vi "Actor Core.vi"(8 "error in (no error)":errorcluster, 11 "Operator UI.lvclass":refnum<class "Measurement UI.lvclass">) -> (0 "error out":errorcluster, 3 "Actor Framework.lvlib:Actor":refnum<class "Actor.lvclass">)   [LabVIEW 2017, in "Measurement UI.lvlib" / "Measurement UI.lvclass"]
doc: "This is Actor Core.vi, the main message handling loop for Actors. An actor usually just sits in this loop and processes messages as they arrive. Any error returned by the message Do.vi call will stop the loop, with error code 43 as the cannonical signal to stop with no error sent to caller. Descendants may override that in Handle Error.vi."
uses:
  Measurement UI.lvclass
  <vilib>/ActorFramework/Actor/Actor.lvclass
  \\Mac\Home/Documents/MAL-Framework/user.lib/Common Components/User Interface/UI.lvclass
  C:/Program Files (x86)/National Instruments/LabVIEW 2017/vi.lib/ActorFramework/Actor/Actor.lvclass
  <vilib>/ActorFramework/Actor/Actor.lvclass/Actor.ctl
  <vilib>/ActorFramework/Message Enqueuer/Message Enqueuer.lvclass/Message Enqueuer.ctl
  <vilib>/ActorFramework/Message Enqueuer/Init from Existing Queue.vi
  <vilib>/ActorFramework/Message Enqueuer/Enqueue.vi
  <vilib>/ActorFramework/Stop Msg/Stop Msg.lvclass
  C:/Program Files (x86)/National Instruments/LabVIEW 2017/vi.lib/ActorFramework/Message/Message.lvclass
  Messages/Ask Controller to Launch Results UI Msg/Ask Controller to Launch Results UI Msg.lvclass
  Measurement UI Messages/Launch Step Configuration Msg/Launch Step Configuration Msg.lvclass
  Accessors/Write Digitizer.vi
  Accessors/Write Function Generator.vi
  Accessors/Write Load New Measurement.vi
  Accessors/Write Measurement.vi
  Accessors/Write Multimeter.vi
  Accessors/Write Power Supply.vi
  Accessors/Write Results Listbox.vi
  Accessors/Write Run.vi
  Accessors/Write Show FP_.vi
  Accessors/Write Status Display.vi
  Accessors/Write Stop Button.vi
  Accessors/Write Tab Control.vi
  Accessors/Write View Results.vi
  Write Step Iterations.vi
  Write settings button array for hardware.vi
  Accessors/Write Step Config.vi
  <vilib>/ActorFramework/Message Priority Queue/Priority Enqueue.vi
  <vilib>/ActorFramework/Message Enqueuer/Message Enqueuer.lvclass
  User Interface/UI.lvclass
  Messages/Send Run Measurement Message/Send Run Measurement Message.lvclass
  Messages/Send Get Hardware Info Message/Send Get Hardware Info Message.lvclass
  Messages/Check Run Button/Check Validity of Selection.lvclass
  Messages/Prompt User for Path to load/Prompt User for File Path to Load From.lvclass
  Measurement UI Messages/Launch Hardware Settings Msg/Launch Hardware Settings Msg.lvclass
panel:
  in  "Step Config":bool
  in  "3":bool
  in  "2":bool
  in  "1":bool
  in  "0":bool
  in  "Step Iterations":i32
  in  "Indefinite run":bool
  in  "about":bool
  in  "Load New Measurement":bool
  in  "Show FP?":bool
  in  "Stop Button":bool
  in  "Run":bool
  in  "Device 4":u16(ring)
  in  "Device 3":u16(ring)
  in  "Device 2":u16(ring)
  in  "Device 1":u16(ring)
  in  "Tab Control":enum32{"Test Status", "Results"}(tab)
  in  "Status Display":string
  in  "View Results":bool
  in  "Results Listbox":i32(listbox)
  in  "Step":u16(ring)
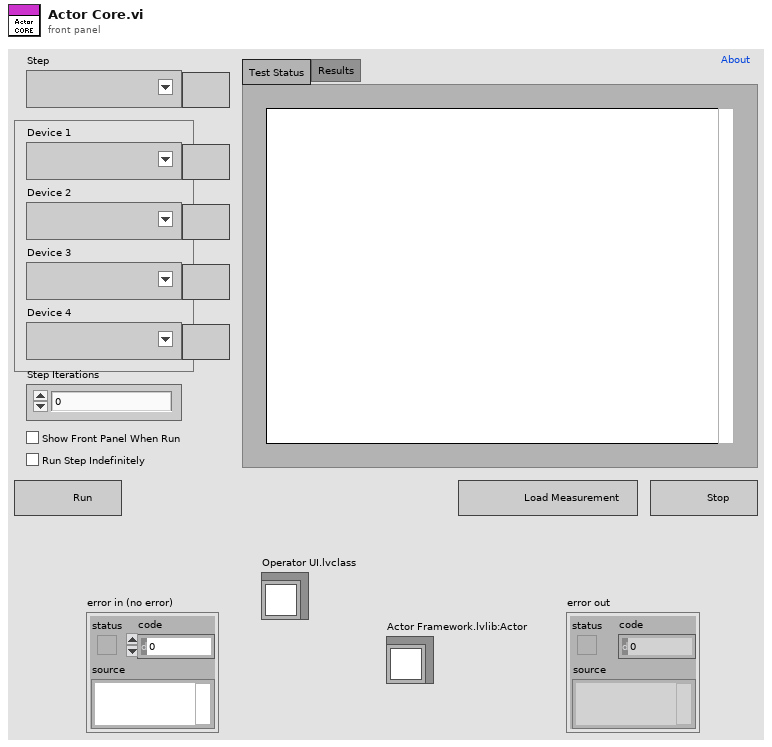
[diagram p1: front panel]
types:
  T1 = enum8{"Enabled", "Disabled", "Disabled and Grayed Out"}
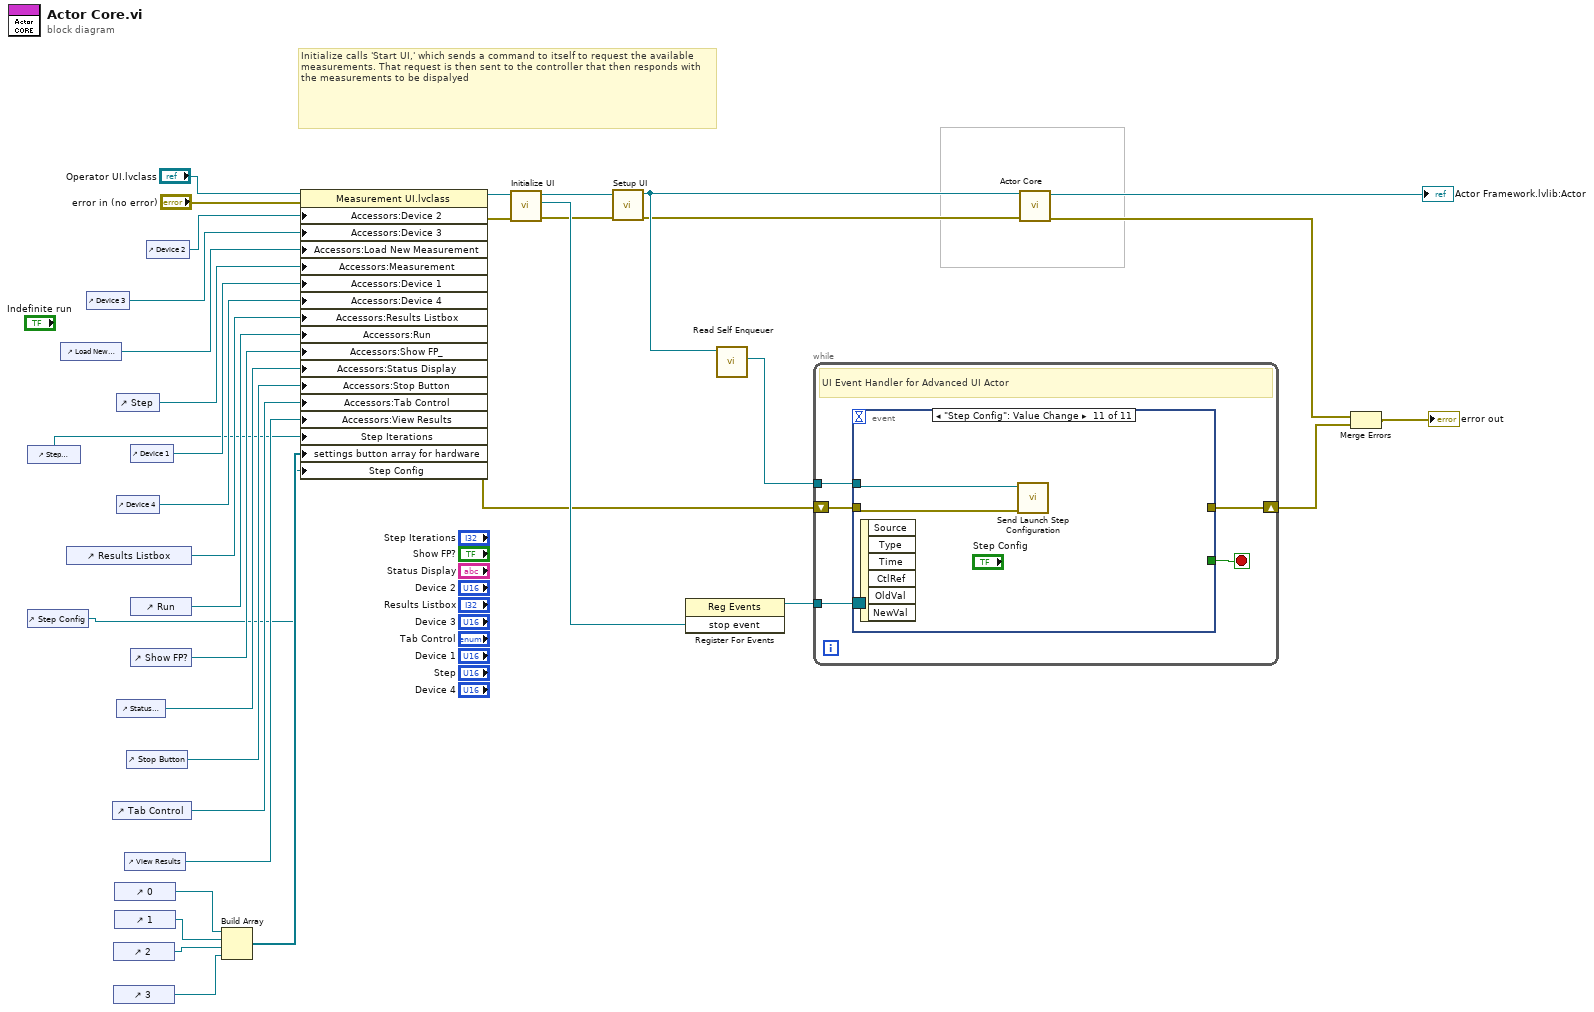
[diagram p0: block diagram]
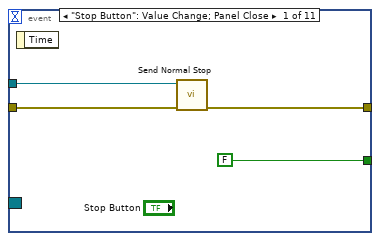
[diagram p2: hidden frame]
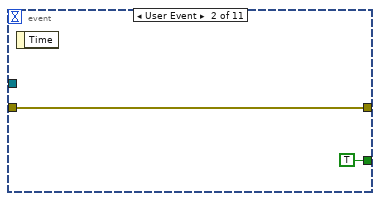
[diagram p3: hidden frame]
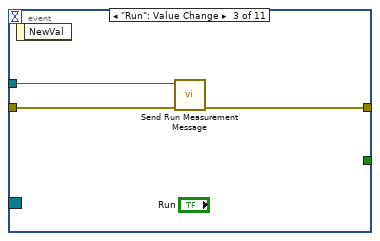
[diagram p4: hidden frame]
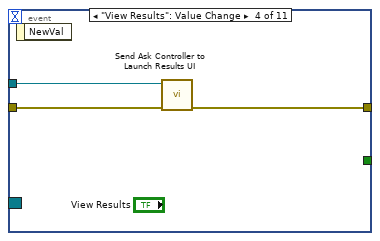
[diagram p5: hidden frame]
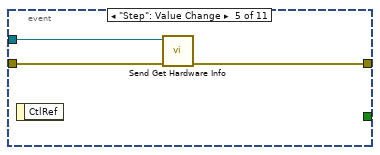
[diagram p6: hidden frame]
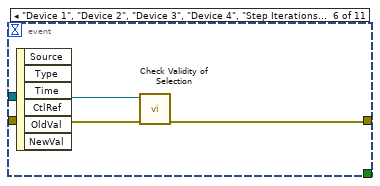
[diagram p7: hidden frame]
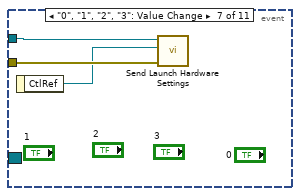
[diagram p8: hidden frame]
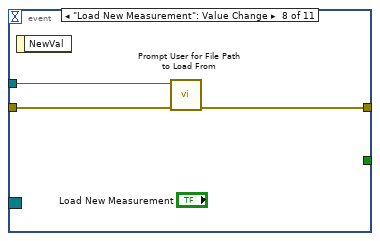
[diagram p9: hidden frame]
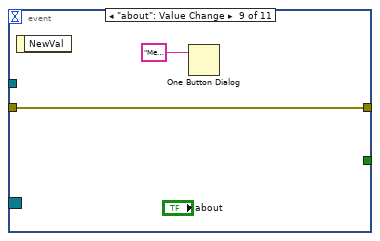
[diagram p10: hidden frame]
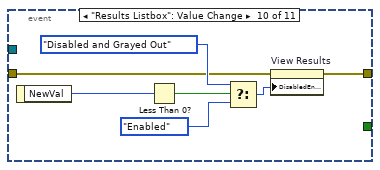
[diagram p11: hidden frame]
diagram:
  # "Initialize calls 'Start UI,' which sends a command to itself to request the available measurements. That request is then sent to the controller that then responds with the measurements to be dispalyed"
  n1 = control-ref of="Step Iterations"() -> (w7:refnum<vi>)
  n2 = control-ref of="Step Config"() -> (w1:refnum<vi>)
  n3 = control-ref of="Load New Measurement"() -> (w18:refnum<vi>)
  n4 = control-ref of="Results Listbox"() -> (w22:refnum<vi>)
  n5 = control-ref of="Device 3"() -> (w19:refnum<vi>)
  n6 = control-ref of="Tab Control"() -> (w24:refnum<vi>)
  n7 = control-ref of="2"() -> (w4:refnum<vi>)
  n8 = control-ref of="3"() -> (w3:refnum<vi>)
  n9 = control-ref of="0"() -> (w6:refnum<vi>)
  n10 = control-ref of="1"() -> (w5:refnum<vi>)
  n11 = control-ref of="Step"() -> (w17:refnum<vi>)
  n12 = control-ref of="Device 4"() -> (w21:refnum<vi>)
  n13 = control-ref of="Status Display"() -> (w26:refnum<vi>)
  n14 = control-ref of="View Results"() -> (w23:refnum<vi>)
  n15 = control-ref of="Stop Button"() -> (w25:refnum<vi>)
  n16 = control-ref of="Device 1"() -> (w16:refnum<vi>)
  n17 = control-ref of="Run"() -> (w15:refnum<vi>)
  n18 = control-ref of="Show FP?"() -> (w27:refnum<vi>)
  n19 = control-ref of="Device 2"() -> (w20:refnum<vi>)
  n20 = Build Array(w6, w5, w4, w3) -> (w2:refnum<vi>[])
  n21 = property class="Measurement UI.lvclass"(reference="Operator UI.lvclass", error in="error in (no error)", "Accessors:Device 2"=w20, "Accessors:Device 3"=w19, "Accessors:Load New Measurement"=w18, "Accessors:Measurement"=w17, "Accessors:Device 1"=w16, "Accessors:Device 4"=w21, "Accessors:Results Listbox"=w22, "Accessors:Run"=w15, "Accessors:Show FP_"=w27, "Accessors:Status Display"=w26, "Accessors:Stop Button"=w25, "Accessors:Tab Control"=w24, "Accessors:View Results"=w23, "Step Iterations"=w7, "settings button array for hardware"=w2, "Step Config"=w1) -> (reference out=w13:refnum<class "Measurement UI.lvclass">, error out=w10:errorcluster)
  n22 = call "Initialize UI.vi"("error in (no error)"=w10, "UI in"=w13) -> ("error out"=w11:errorcluster, "stop event"=w29:refnum<user-event>, "UI out"=w12:refnum<class "Measurement UI.lvclass">)  [unwired: 7 in]
  n23 = call-dynamic "Setup UI.vi"("error in (no error)"=w11, "Operator UI in"=w12) -> ("error out"=w8:errorcluster, "Operator UI out"=w9:refnum<class "Measurement UI.lvclass">)  [unwired: 8 in]
  n24 = register-events(w29) -> (reference out=w30:refnum<event-registration>)  [unwired: 2 in, 1 out]
  n25 = call <vilib>:"Read Self Enqueuer.vi"("Actor"=w9) -> ("Self Enqueuer"=w34:refnum<class "Message Enqueuer.lvclass">)  [unwired: 10 in]
  n26 = while {
    tunnel: w34 -> [w39]
    tunnel: w30 -> [w38]
    shift-right: [w36] -> w33
    shift-left: w10 -> [w37]
    stop <- w40 stop-if-true
    # "UI Event Handler for Advanced UI Actor"
    n27 = event shown="[10] \"Step Config\": Value Change" {
      selector: w38 -> [_ _ _ _ _ _ _ _ _ _ _]
      dyn-events: _ -> [_ _ _ _ _ _ _ _ _ _ _]
      timeout: _ -> [_ _ _ _ _ _ _ _ _ _ _]
      tunnel: [FALSE TRUE _ _ _ _ _ _ _ _ _] -> w40
      tunnel: w39 -> [w43 _ w49 w52 w55 w58 w61 w64 _ _ w75]
      tunnel: w37 -> [w42 w45 w48 w51 w54 w57 w60 w63 w65 w68 w74]
      tunnel: [w41 w45 w47 w50 w53 w56 _ w62 w65 w67 _] -> w36
      event "Stop Button": Value Change; Panel Close {
        n28 = event-data() -> ()  [unwired: 1 in, 1 out]
        n29 = call <vilib>:"Send Normal Stop.vi"("error in (no error)"=w42, "Message Enqueuer"=w43) -> ("error out"=w41:errorcluster)  [unwired: 9 in]
      }
      event User Event {
        n30 = event-data() -> ()  [unwired: 1 in, 1 out]
      }
      event "Run": Value Change {
        n31 = event-data() -> ()  [unwired: 1 in, 1 out]
        n32 = call "Send Run Measurement Message.vi"("error in (no error)"=w48, "Message Enqueuer in"=w49) -> ("error out"=w47:errorcluster)  [unwired: 8 in, 1 out]
      }
      event "View Results": Value Change {
        n33 = event-data() -> ()  [unwired: 1 in, 1 out]
        n34 = call "Send Ask Controller to Launch Results UI.vi"("error in (no error)"=w51, "Message Enqueuer in"=w52) -> ("error out"=w50:errorcluster)  [unwired: 8 in, 1 out]
      }
      event "Step": Value Change {
        n35 = event-data() -> ()  [unwired: 1 in, 1 out]
        n36 = call "Send Get Hardware Info.vi"("error in (no error)"=w54, "Message Enqueuer in"=w55) -> ("error out"=w53:errorcluster)  [unwired: 8 in, 1 out]
      }
      event "Device 1", "Device 2", "Device 3", "Device 4", "Step Iterations", "Indefinite run": Value Change {
        n37 = event-data() -> ()  [unwired: 1 in, 6 out]
        n38 = call "Check Validity of Selection.vi"("error in (no error)"=w57, "Message Enqueuer in"=w58) -> ("error out"=w56:errorcluster)  [unwired: 8 in, 1 out]
      }
      event "0", "1", "2", "3": Value Change {
        n39 = event-data() -> ("CtlRef"=w59:refnum<vi>)  [unwired: 1 in]
        n40 = call "Send Launch Hardware Settings.vi"("error in (no error)"=w60, "button ref"=w59, "Message Enqueuer"=w61) -> ()  [unwired: 7 in, 2 out]
      }
      event "Load New Measurement": Value Change {
        n41 = event-data() -> ()  [unwired: 1 in, 1 out]
        n42 = call "Prompt User for File Path to Load From.vi"("error in (no error)"=w63, "Message Enqueuer in"=w64) -> ("error out"=w62:errorcluster)  [unwired: 8 in, 1 out]
      }
      event "about": Value Change {
        n43 = event-data() -> ()  [unwired: 1 in, 1 out]
        n44 = One Button Dialog(message="Measurement Manager v2.0\n\nNational Instruments (C) 2013\nWritten in NI LabVIEW 2012 by Elijah Kerry \nElijah.Kerry@ni.com\n\nni.com/largeapps\nekerry.wordpress.com") -> ()  [unwired: 1 in, 1 out]
      }
      event "Results Listbox": Value Change {
        n45 = event-data() -> ("NewVal"=w69:i32)  [unwired: 1 in]
        n46 = Less Than 0?(x=w69) -> (x < 0?=w70:bool)
        n47 = Select(t=T1."Disabled and Grayed Out" ("Disabled"), s=w70, f=T1."Enabled" ("Disabled")) -> (s? t:f=w73:T1)
        n48 = property on="View Results" class="Bool"(error in=w68, "DisabledEnum"=w73) -> (error out=w67:errorcluster)  [unwired: 1 in, 1 out]
      }
      event "Step Config": Value Change {
        n49 = event-data() -> ()  [unwired: 1 in, 6 out]
        n50 = call "Send Launch Step Configuration.vi"("error in (no error)"=w74, "Message Enqueuer"=w75) -> ()  [unwired: 8 in, 2 out]
      }
    }
  }
  n51 = call-parent "Actor Core.vi"("error in"=w8, "User Interface"=w9) -> ("error out"=w32:errorcluster, "Actor out"=→"Actor Framework.lvlib:Actor":refnum<class "Actor.lvclass">)  [unwired: 8 in]
  n52 = Merge Errors(w32, w33) -> (→"error out":errorcluster)
